vi "Compile APU 1.4 Data.vi"(8 "error in (no error)":errorcluster, 11 "Device Item Ref in":T3 format="%.0x") -> (0 "error out":errorcluster, 2 "APUs":T1[](array[typedef]), 3 "Device Item Ref out":T3 format="%.0x")   [LabVIEW 2020, in "Engine Simulation Toolkit System Explorer.lvlib"]
uses:
  Engine Simulation Toolkit System Explorer.lvlib
  <vilib>/NI VeriStand/Custom Device API/Custom Device Item Ref.ctl
  Shared/1.4 APU Engine Data.ctl
  Shared/1.4 APU Engine FIFO Idxs.ctl
  Shared/Properties.vi
  Shared/Constants and GUIDs.vi
  <vilib>/NI VeriStand/Custom Device Tools/Custom Device Utility Library/NI VeriStand - Search for All Items by GUID.vi
  <vilib>/NI VeriStand/Custom Device API/Get Item Property (String).vi
  <vilib>/NI VeriStand/Custom Device API/Get Item Property (Double).vi
  <vilib>/NI VeriStand/Custom Device API/Get Item Property (Boolean).vi
  <vilib>/NI VeriStand/Custom Device API/Get Item Property (U16).vi
  <vilib>/NI VeriStand/Custom Device Tools/Custom Device Utility Library/NI VeriStand - Search for Item by GUID.vi
  Shared/Engine Simulation Toolkit Shared.lvlib
  <vilib>/NI VeriStand/Custom Device API/Custom Device API.lvlib
  <vilib>/NI VeriStand/Custom Device Tools/Custom Device Utility Library/Custom Device Utility Library.lvlib
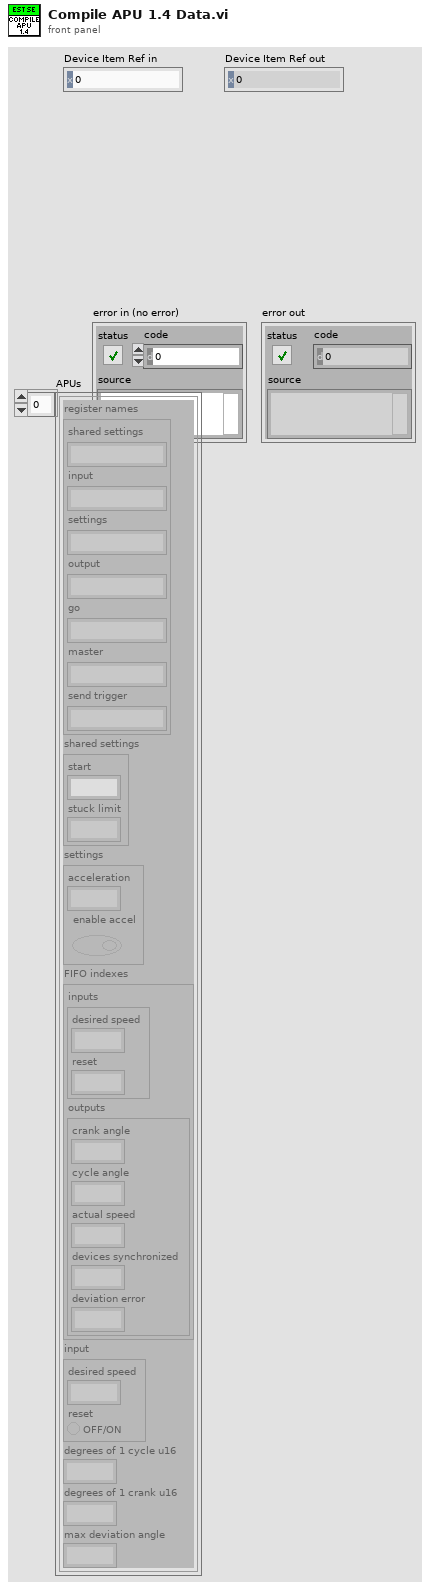
[diagram p1: front panel]
types:
  T1 = typedef "Engine Simulation Toolkit Shared.lvlib/1.4 APU Engine Data.ctl" = cluster{"register names":cluster{"shared settings":string, "input":string, "settings":string, "output":string, "go":string, "master":string, "send trigger":string}, "shared settings":cluster{"start":fxp<+,17,17>, "stuck limit":fxp<+,18,18>}, "settings":cluster{"acceleration":fxp<+,18,-20>, "enable accel":bool}, "FIFO indexes":T2, "input":cluster{"desired speed":fxp<+/-,23,2>, "reset":bool}, "degrees of 1 cycle u16":dbl, "degrees of 1 crank u16":dbl, "max deviation angle":dbl}
  T2 = typedef "Engine Simulation Toolkit Shared.lvlib/1.4 APU Engine FIFO Idxs.ctl" = cluster{"inputs":cluster{"desired speed":i32, "reset":i32}, "outputs":cluster{"crank angle":i32, "cycle angle":i32, "actual speed":i32, "devices synchronized":i32, "deviation error":i32}}
  T3 = typedef "Custom Device API.lvlib/Custom Device Item Ref.ctl" = u64
  T4 = typedef "Engine Simulation Toolkit Shared.lvlib/Channel.ctl" = cluster{"Name":string, "Units":string, "Default":dbl, "Description":string, "Scalable":bool}
  T5 = cluster{"desired speed":fxp<+/-,23,2>, "reset":bool}
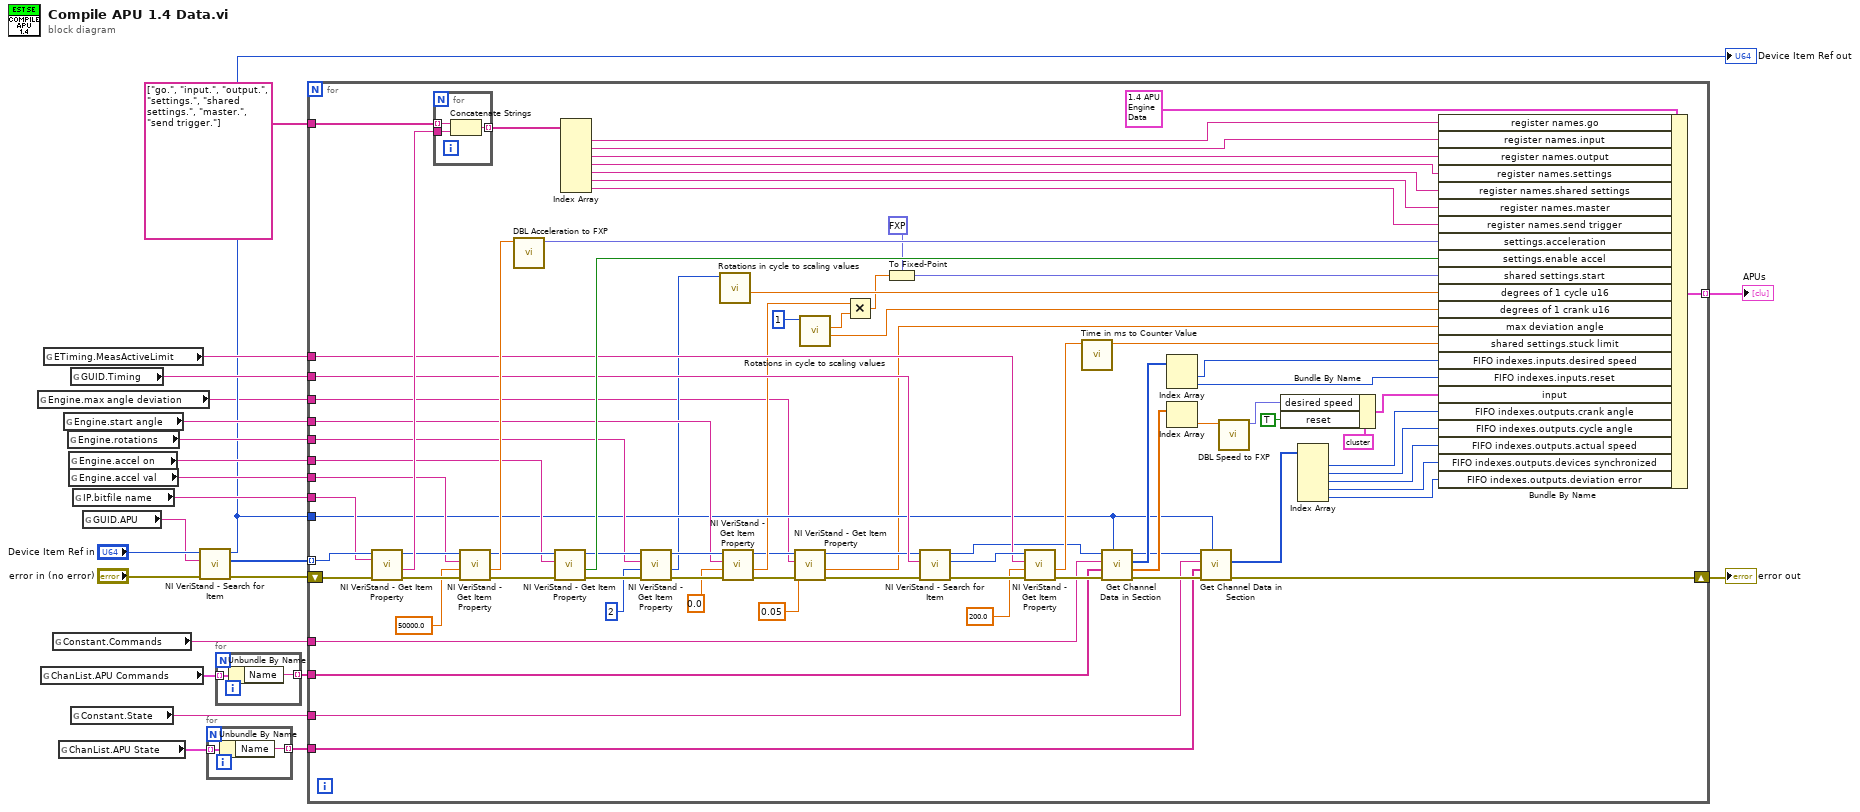
[diagram p0: block diagram]
diagram:
  n1 = global read "Properties.vi" "Engine.max angle deviation"() -> (w1:string)
  n2 = global read "Constants and GUIDs.vi" "ChanList.APU Commands"() -> (w7:T4[])
  n3 = global read "Properties.vi" "ETiming.MeasActiveLimit"() -> (w11:string)
  n4 = global read "Constants and GUIDs.vi" "Constant.Commands"() -> (w10:string)
  n5 = global read "Constants and GUIDs.vi" "ChanList.APU State"() -> (w5:T4[])
  n6 = global read "Properties.vi" "Engine.start angle"() -> (w13:string)
  n7 = global read "Properties.vi" "Engine.rotations"() -> (w14:string)
  n8 = global read "Properties.vi" "Engine.accel on"() -> (w15:string)
  n9 = global read "Properties.vi" "Engine.accel val"() -> (w17:string)
  n10 = global read "Constants and GUIDs.vi" "GUID.Timing"() -> (w12:string)
  n11 = global read "Constants and GUIDs.vi" "Constant.State"() -> (w8:string)
  n12 = global read "Properties.vi" "IP.bitfile name"() -> (w19:string)
  n13 = global read "Constants and GUIDs.vi" "GUID.APU"() -> (w21:string)
  n14 = call-poly <vilib>:"NI VeriStand - Search for Item.vi"("error in"="error in (no error)", "Item GUID"=w21, "Section Ref in"="Device Item Ref in") -> ("error out"=w20:errorcluster, "Item Refs"=w3:T3[], "Section Ref out"=w9:T3)  [unwired: 5 in, 1 out]
  "Device Item Ref out" <- w9
  n15 = for {
    tunnel: w5 -> [w25] mode=indexing
    tunnel: [w24] -> w4 mode=indexing
    n16 = Unbundle By Name(w25) -> ("Name"=w24:string)
  }
  n17 = for {
    tunnel: w7 -> [w27] mode=indexing
    tunnel: [w26] -> w6 mode=indexing
    n18 = Unbundle By Name(w27) -> ("Name"=w26:string)
  }
  n19 = for {
    shift-right: [w64] -> w16
    shift-left: w20 -> [w108]
    tunnel: w3 -> [w107] mode=indexing
    tunnel: w19 -> [w106]
    tunnel: string[] ["go.", "input.", "output.", "settings.", "shared settings.", "master.", "send trigger."] -> [w104]
    tunnel: w17 -> [w99]
    tunnel: w15 -> [w93]
    tunnel: w14 -> [w89]
    tunnel: w13 -> [w86]
    tunnel: w12 -> [w83]
    tunnel: w11 -> [w80]
    tunnel: w10 -> [w75]
    tunnel: w6 -> [w53]
    tunnel: [w69] -> w2 mode=indexing
    tunnel: w9 -> [w63]
    tunnel: w8 -> [w61]
    tunnel: w4 -> [w52]
    tunnel: w1 -> [w31]
    n20 = call-poly <vilib>:"NI VeriStand - Get Item Property.vi"("error in (no error)"=w108, "Property Name"=w106, "Item Ref in"=w107) -> ("error out"=w100:errorcluster, "Value"=w105:string, "Item Ref out"=w101:T3)  [unwired: 5 in, 1 out]
    n21 = for {
      tunnel: w105 -> [w111]
      tunnel: w104 -> [w110] mode=indexing
      tunnel: [w109] -> w102 mode=indexing
      n22 = Concatenate Strings(w110, w111) -> (w109:string)
    }
    n23 = call-poly <vilib>:"NI VeriStand - Get Item Property.vi"("error in (no error)"=w100, "Default Value"=50000.0, "Property Name"=w99, "Item Ref in"=w101) -> ("error out"=w98:errorcluster, "Value"=w97:dbl, "Item Ref out"=w94:T3)  [unwired: 4 in, 1 out]
    n24 = call "DBL Acceleration to FXP.vi"("Desired acceleration (RPM/sec)"=w97) -> ("FXP acceleration"=w96:fxp<+,18,-20>)  [unwired: 6 in, 4 out]
    n25 = call-poly <vilib>:"NI VeriStand - Get Item Property.vi"("error in (no error)"=w98, "Property Name"=w93, "Item Ref in"=w94) -> ("error out"=w95:errorcluster, "Value"=w92:bool, "Item Ref out"=w90:T3)  [unwired: 5 in, 1 out]
    n26 = Index Array(array=w102) -> (element #1=w51:string, element #2=w50:string, element #3=w49:string, element #4=w48:string, element #5=w47:string, element #6=w29:string, element #7=w28:string)  [unwired: 7 in]
    n27 = call-poly <vilib>:"NI VeriStand - Get Item Property.vi"("error in (no error)"=w95, "Default Value"=u16 2, "Property Name"=w89, "Item Ref in"=w90) -> ("error out"=w91:errorcluster, "Value"=w46:u16, "Item Ref out"=w87:T3)  [unwired: 4 in, 1 out]
    n28 = call "Rotations in cycle to scaling values.vi"("rotations in a cycle"=w46) -> ("degrees of one u16"=w45:dbl)  [unwired: 8 in, 2 out]
    n29 = call-poly <vilib>:"NI VeriStand - Get Item Property.vi"("error in (no error)"=w91, "Default Value"=0.0, "Property Name"=w86, "Item Ref in"=w87) -> ("error out"=w35:errorcluster, "Value"=w43:dbl, "Item Ref out"=w37:T3)  [unwired: 4 in, 1 out]
    n30 = call-poly <vilib>:"NI VeriStand - Get Item Property.vi"("error in (no error)"=w35, "Default Value"=0.05, "Property Name"=w31, "Item Ref in"=w37) -> ("error out"=w34:errorcluster, "Value"=w32:dbl, "Item Ref out"=w33:T3)  [unwired: 4 in, 1 out]
    n31 = call "Rotations in cycle to scaling values.vi"("rotations in a cycle"=u16 1) -> ("degrees of one u16"=w54:dbl, "angle to u16 scale factor"=w44:dbl)  [unwired: 8 in, 1 out]
    n32 = Multiply(x=w43, y=w44) -> (x*y=w42:dbl)
    n33 = To Fixed-Point(fixed-point type=fxp<+,17,17> 0.0 ("shared settings.start"), number=w42) -> (fixed-point=w40:fxp<+,17,17>)
    n34 = call-poly <vilib>:"NI VeriStand - Search for Item.vi"("error in"=w34, "Item GUID"=w83, "Section Ref in"=w33) -> ("error out"=w84:errorcluster, "Item Ref"=w81:T3, "Section Ref out"=w76:T3)  [unwired: 5 in, 1 out]
    n35 = call-poly <vilib>:"NI VeriStand - Get Item Property.vi"("error in (no error)"=w84, "Default Value"=200.0, "Property Name"=w80, "Item Ref in"=w81) -> ("error out"=w82:errorcluster, "Value"=w78:dbl)  [unwired: 4 in, 2 out]
    n36 = call "Time in ms to Counter Value.vi"("time (ms)"=w78) -> ("counter value"=w77:dbl)  [unwired: 10 in]
    n37 = call "Get Channel Data in Section.vi"("Custom device ref"=w63, "error in (no error)"=w82, "Channels"=w53, "Section (\"\":none)"=w75, "Item Ref in"=w76) -> ("error out"=w74:errorcluster, "default values"=w68:dbl[], "FIFO indexes"=w73:i32[], "Item Ref out"=w62:T3)  [unwired: 2 in, 1 out]
    n38 = Index Array(array=w73) -> (element #1=w72:i32, element #2=w71:i32)  [unwired: 2 in]
    n39 = Index Array(array=w68) -> (element=w67:dbl)  [unwired: 1 in]
    n40 = call "Get Channel Data in Section.vi"("Custom device ref"=w63, "error in (no error)"=w74, "Channels"=w52, "Section (\"\":none)"=w61, "Item Ref in"=w62) -> ("error out"=w64:errorcluster, "FIFO indexes"=w60:i32[])  [unwired: 2 in, 3 out]
    n41 = call "DBL Speed to FXP.vi"("Desired speed (RPM)"=w67) -> ("FXP speed"=w65:fxp<+/-,23,2>)  [unwired: 6 in, 4 out]
    n42 = Bundle By Name(cluster=T5 {"desired speed"=0.0, "reset"=FALSE} ("input"), "desired speed"=w65, "reset"=TRUE) -> (w66:T5)
    n43 = Index Array(array=w60) -> (element #1=w59:i32, element #2=w58:i32, element #3=w57:i32, element #4=w38:i32, element #5=w39:i32)  [unwired: 5 in]
    n44 = Bundle By Name(cluster=T1 {"register names"={"shared settings"="", "input"="", "settings"="", "output"="", "go"="", "master"="", "send trigger"=""}, "shared settings"={"start"=0.0, "stuck limit"=0.0}, "settings"={"acceleration"=0.0, "enable accel"=FALSE}, "FIFO indexes"={"inputs"={"desired speed"=0, "reset"=0}, "outputs"={"crank angle"=0, "cycle angle"=0, "actual speed"=0, "devices synchronized"=0, "deviation error"=0}}, "input"={"desired speed"=0.0, "reset"=FALSE}, "degrees of 1 cycle u16"=0.0, "degrees of 1 crank u16"=0.0, "max deviation angle"=0.0} ("1.4.0 APU"), "register names.go"=w51, "register names.input"=w50, "register names.output"=w49, "register names.settings"=w48, "register names.shared settings"=w47, "register names.master"=w29, "register names.send trigger"=w28, "settings.acceleration"=w96, "settings.enable accel"=w92, "shared settings.start"=w40, "degrees of 1 cycle u16"=w45, "degrees of 1 crank u16"=w54, "max deviation angle"=w32, "shared settings.stuck limit"=w77, "FIFO indexes.inputs.desired speed"=w72, "FIFO indexes.inputs.reset"=w71, "input"=w66, "FIFO indexes.outputs.crank angle"=w59, "FIFO indexes.outputs.cycle angle"=w58, "FIFO indexes.outputs.actual speed"=w57, "FIFO indexes.outputs.devices synchronized"=w38, "FIFO indexes.outputs.deviation error"=w39) -> (w69:T1)
  }
  "error out" <- w16
  "APUs" <- w2
